vi "RemoteVI Greeting.vi"(0 "VI name":string, 1 "view only?":bool) -> (4 "hello":string)   [LabVIEW 2020, in "RemoteVI.lvlib"]
doc: "The frames every new client gets first (docs\\protocol.md): the text messages \"title <VI name>\" and \"viewonly 0\" (1 with view only? TRUE), each as a WebSocket text frame (RemoteVI WS Encode Server Frame.vi), concatenated. Pure."
uses:
  RemoteVI.lvlib
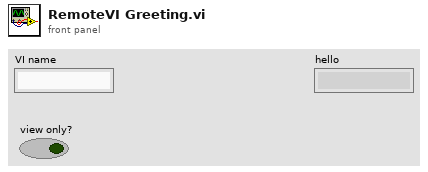
[diagram p1: front panel]
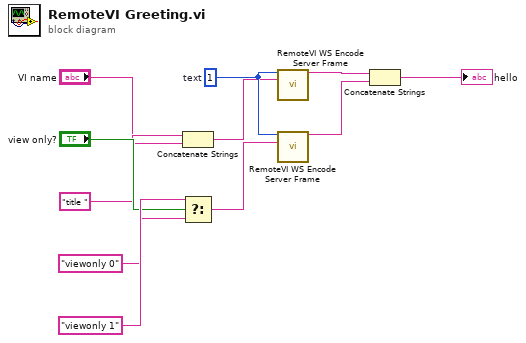
[diagram p0: block diagram]
diagram:
  w4 = u8 1  # text
  n1 = Concatenate Strings("title ", "VI name") -> (w3:string)
  n2 = Select(t="viewonly 1", s="view only?", f="viewonly 0") -> (s? t:f=w8:string)
  n3 = call "RemoteVI WS Encode Server Frame.vi"("opcode"=w4, "payload"=w3) -> ("frame"=w9:string)  [unwired: 13 in]
  n4 = call "RemoteVI WS Encode Server Frame.vi"("opcode"=w4, "payload"=w8) -> ("frame"=w10:string)  [unwired: 13 in]
  n5 = Concatenate Strings(w9, w10) -> (→"hello":string)
